vi "Replace Line.vi"(8 "error in":errorcluster, 9 "New Line":T1, 10 "Line Name":string, 11 "tag bus configurable plugin module configuration in":refnum<class "tag bus configurable plugin module configuration.lvclass">) -> (0 "error out":errorcluster, 2 "Old Line":T1, 3 "tag bus configurable plugin module configuration out":refnum<class "tag bus configurable plugin module configuration.lvclass">)   [LabVIEW 2014, in "tag bus configurable plugin module configuration.lvclass"]
uses:
  tag bus configurable plugin module configuration.lvclass
  Line.ctl
  <vilib>/NI/Tag Bus Module Framework/channel/TBM channel.lvclass
  tag bus configurable plugin module configuration.lvclass/tag bus configurable plugin module configuration.ctl
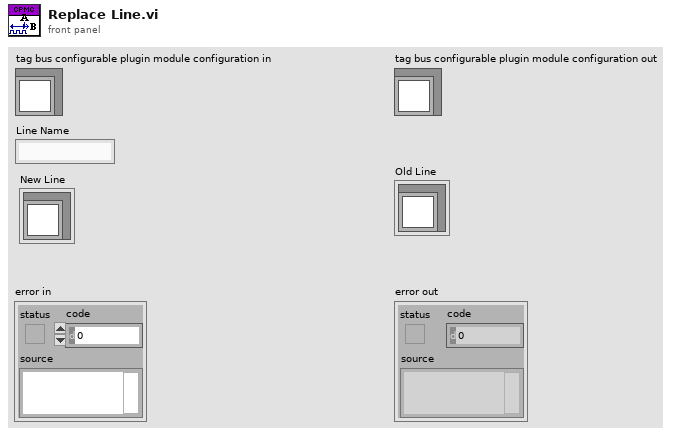
[diagram p1: front panel]
types:
  T1 = typedef "tag bus configurable plugin module configuration.lvclass/Line.ctl" = cluster{"channel":refnum<class "TBM channel.lvclass">}
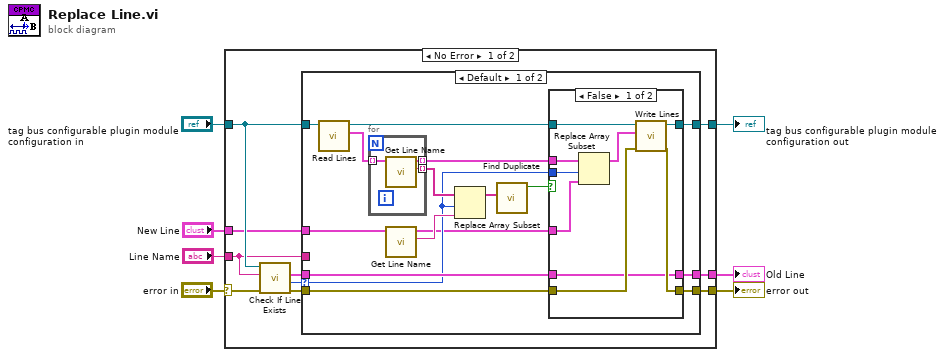
[diagram p0: block diagram]
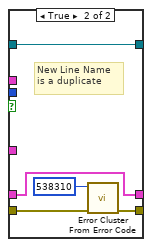
[diagram p2: hidden frame]
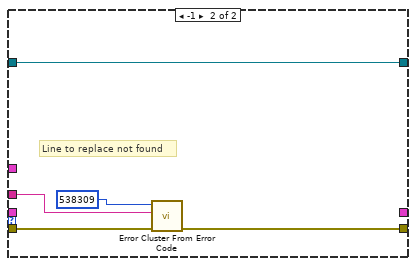
[diagram p3: hidden frame]
diagram:
  n1 = case shown="No Error" "error in" {
    selector: "error in" -> [w10 w57]
    tunnel: [w16 w57] -> w6
    tunnel: [w17 w56] -> w4
    tunnel: "tag bus configurable plugin module configuration in" -> [w15 w56]
    tunnel: "Line Name" -> [w14 _]
    tunnel: "New Line" -> [w12 _]
    tunnel: [w11 _] -> w1
    frame No Error {
      n2 = call-dynamic "Check If Line Exists.vi"("error in"=w10, "name to locate"=w14, "tag bus configurable plugin module configuration in"=w15) -> ("error out"=w9:errorcluster, "index"=w13:i32, "Line out"=w8:T1)  [unwired: 4 in, 2 out]
      n3 = case shown="Default" w13 {
        selector: w13 -> [w20 _]
        tunnel: w15 -> [w33 w55]
        tunnel: [w18 w55] -> w17
        tunnel: w12 -> [w23 _]
        tunnel: w14 -> [_ w53]
        tunnel: w9 -> [w28 w52]
        tunnel: [w27 w51] -> w16
        tunnel: [w26 _] -> w11
        tunnel: w8 -> [w25 _]
        frame Default {
          n4 = call "Read Lines.vi"("tag bus configurable plugin module configuration in"=w33) -> ("Lines"=w30:T1[], "tag bus configurable plugin module configuration out"=w32:refnum<class "tag bus configurable plugin module configuration.lvclass">)  [unwired: 8 in, 1 out]
          n5 = for {
            tunnel: w30 -> [w36] mode=indexing
            tunnel: [w35] -> w29 mode=indexing
            tunnel: [w34] -> w22 mode=indexing
            n6 = call "Get Line Name.vi"("Line in"=w36) -> ("Name"=w34:string, "Line out"=w35:T1)  [unwired: 8 in, 1 out]
          }
          n7 = call "Get Line Name.vi"("Line in"=w23) -> ("Name"=w24:string, "Line out"=w19:T1)  [unwired: 8 in, 1 out]
          n8 = Replace Array Subset(array=w22, new element=w24, index=w20) -> (w31:string[])
          n9 = call "Find Duplicate.vi"("strings"=w31) -> ("duplicate exists"=w21:bool)  [unwired: 8 in, 2 out]
          n10 = case shown="False" w21 {
            tunnel: w32 -> [w42 w46]
            tunnel: w29 -> [w45 _]
            tunnel: w28 -> [w39 w49]
            tunnel: [w38 w48] -> w27
            tunnel: [w37 w47] -> w26
            tunnel: w25 -> [w37 w47]
            tunnel: w20 -> [w44 _]
            tunnel: w19 -> [w43 _]
            tunnel: [w41 w46] -> w18
            frame False {
              n11 = Replace Array Subset(array=w45, new element=w43, index=w44) -> (w40:T1[])
              n12 = call "Write Lines.vi"("error in (no error)"=w39, "Lines"=w40, "tag bus configurable plugin module configuration in"=w42) -> ("error out"=w38:errorcluster, "tag bus configurable plugin module configuration out"=w41:refnum<class "tag bus configurable plugin module configuration.lvclass">)  [unwired: 7 in]
            }
            frame True {
              # "New Line Name is a duplicate"
              n13 = call <vilib>:"Error Cluster From Error Code.vi"("error in (no error)"=w49, "error code (0)"=538310) -> ("error out"=w48:errorcluster)  [unwired: 7 in]
            }
          }
        }
        frame -1 {
          # "Line to replace not found"
          n14 = call <vilib>:"Error Cluster From Error Code.vi"("error in (no error)"=w52, "error message (\"\")"=w53, "error code (0)"=538309) -> ("error out"=w51:errorcluster)  [unwired: 6 in]
        }
      }
    }
    frame Error {
    }
  }
  "error out" <- w6
  "tag bus configurable plugin module configuration out" <- w4
  "Old Line" <- w1
